vi "Initialize TCS Stream.vi"(8 "error in (no error)":errorcluster, 10 "TCS Simulated/Real":bool, 11 "TCS in":refnum<class "TCS.lvclass">) -> (0 "error out":errorcluster, 3 "TCS out":refnum<class "TCS.lvclass">)   [LabVIEW 2018, in "TCS.lvclass"]
uses:
  TCS.lvclass
  TCS.lvclass/TCS.ctl
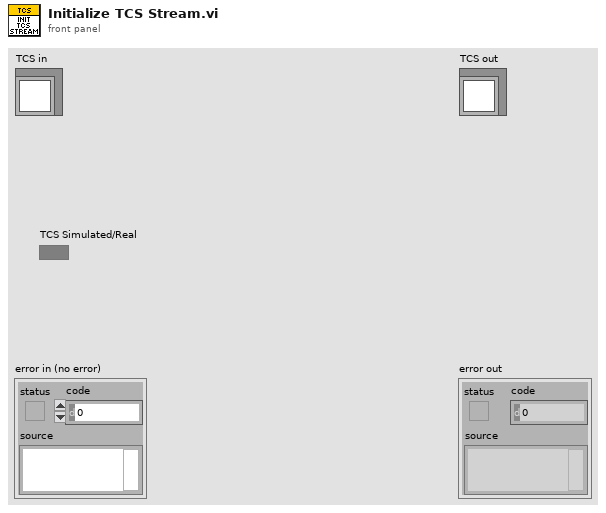
[diagram p1: front panel]
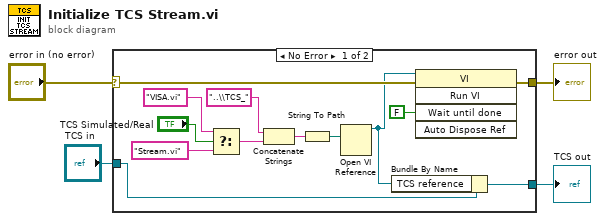
[diagram p0: block diagram]
diagram:
  n1 = case shown="No Error" "error in (no error)" {
    selector: "error in (no error)" -> [w16 w19]
    tunnel: [w15 w19] -> w3
    tunnel: [w13 w18] -> w1
    tunnel: "TCS in" -> [w14 w18]
    frame No Error {
      n2 = Select(t="VISA.vi", s="TCS Simulated/Real", f="Stream.vi") -> (s? t:f=w9:string)
      n3 = Concatenate Strings("..\\TCS_", w9) -> (w6:string)
      n4 = String To Path(string=w6) -> (path=w5:path)
      n5 = Open VI Reference(vi path=w5) -> (vi reference=w12:refnum<vi>)  [unwired: 5 in, 1 out]
      n6 = Bundle By Name(cluster=w14, "TCS reference"=w12) -> (w13:refnum<class "TCS.lvclass">)
      n7 = invoke class="VI" method="Run VI"(reference=w12, error in=w16, "Wait until done"=FALSE ("Wait Until Done")) -> (error out=w15:errorcluster)  [unwired: 2 in, 4 out]
    }
    frame Error {
    }
  }
  "error out" <- w3
  "TCS out" <- w1
